vi "TestArmPathPlanner.vi"() -> ()   [LabVIEW 2017]
uses:
  ArgosLib/Path Planning/TypeDefs/Point2D.ctl
  General/MotionProfiling/TypeDefs/MotionProfileGeneratorParams.ctl
  <vilib>/Rock Robotics/WPI/ThirdParty/Phoenix-LabVIEW/Motor Controller/Controls/CTRE_Phoenix_MotorControl_TrajectoryPointTimeDur.ctl
  TypeDefs/RobotID.ctl
  General/MotionProfiling/TypeDefs/TrajectoryPoint.ctl
panel:
  out "Arm Rotation":T1(graph)
  out "Arm Extension":T1(graph)
  out "Overall Motion":T1(graph)
  out "TravelTime (s)":dbl
  in  "MotionProfileGeneratorParameters":T2={"Trajectory Point Interval (ms)"=40, "Maximum Travel Speed (units/s)"=110.0, "Velocity Ramp Time (ms)"=400.0, "Acceleration Ramp Time (ms)"=200.0} {"Acceleration Ramp Time (ms)" min=1.0; "Velocity Ramp Time (ms)" min=1.0; "Maximum Travel Speed (units/s)" min=0.0; "Trajectory Point Interval (ms)" items=["TrajectoryDuration_0ms"=0, "TrajectoryDuration_5ms"=5, "TrajectoryDuration_10ms"=10, "TrajectoryDuration_20ms"=20, "TrajectoryDuration_30ms"=30, "TrajectoryDuration_40ms"=40, "TrajectoryDuration_50ms"=50, "TrajectoryDuration_100ms"=100]}
  in  "EndPoint":T4={"X"=32.0, "Y"=50.0}
  in  "StartPoint":T4={"X"=32.0, "Y"=-45.0}
  in  "PathPointSpacing (in)":dbl=0.25
  in  "MaxArmLength":dbl=68.0
  in  "MinArmLength":dbl=44.0
  out "PathLength (in)":dbl
  out "NumPoints":i32
  out "Path":cluster{dbl[], dbl[]}[](graph)
  out "Update Rate (Hz)":dbl
  in  "stop":bool
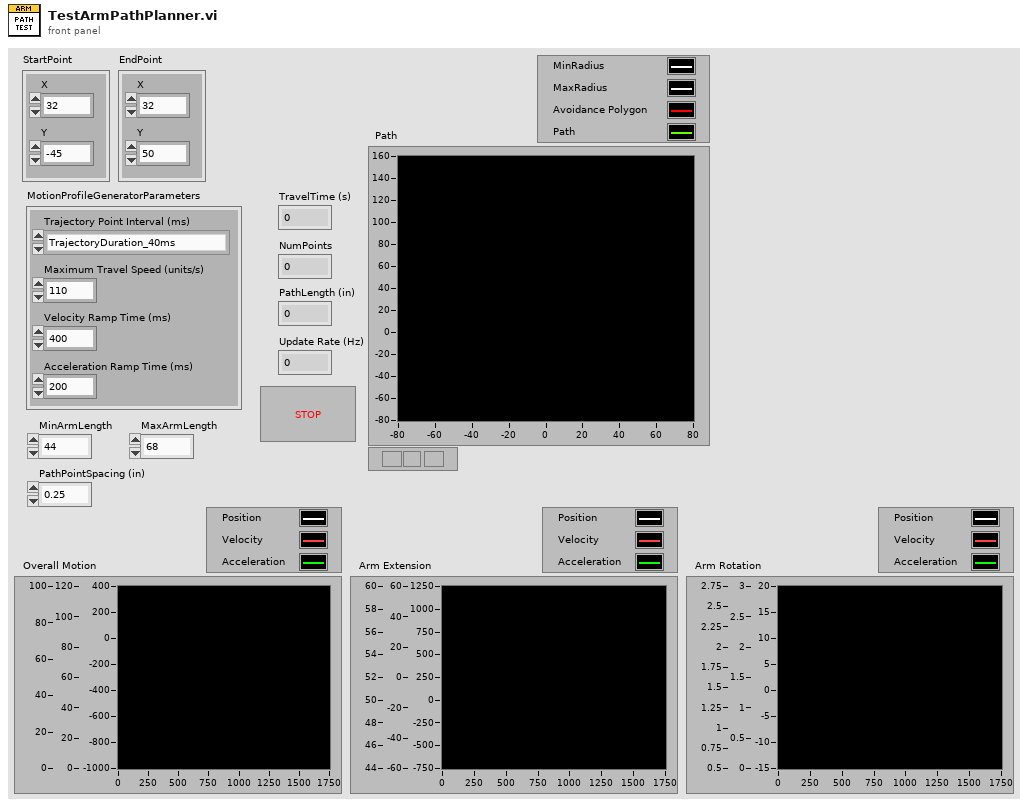
[diagram p1: front panel]
types:
  T1 = cluster{dbl, "Trajectory Point Interval (ms)":i32, dbl[][]}
  T2 = typedef "MotionProfileGeneratorParams.ctl" = cluster{"Trajectory Point Interval (ms)":T3, "Maximum Travel Speed (units/s)":dbl, "Velocity Ramp Time (ms)":dbl, "Acceleration Ramp Time (ms)":dbl}
  T3 = typedef "CTRE_Phoenix_MotorControl_TrajectoryPointTimeDur.ctl" = i32
  T4 = typedef "Point2D.ctl" = cluster{"X":dbl, "Y":dbl}
  T5 = typedef "RobotID.ctl" = enum16{"Competition", "Practice", "Programming", "Demo"}
  T6 = typedef "TrajectoryPoint.ctl" = cluster{"Position ":dbl, "Velocity ":dbl, "Time (ms)":T3, "Last Point":bool}
  T7 = typedef "Config_Robot.ctl" = cluster{"Motors":cluster{"DriveLeftPrimary":T8, "DriveLeftSecondary1":T8, "DriveRightPrimary":T8, "DriveRightSecondary1":T8, "RightIntake":T8, "LeftIntake":T8, "ArmPivot":T8, "ArmExtend":T8, "ArmPivot2":T8, "Climber":T8, "Selfie Stick":T8}, "Sensors":cluster{"IMU":T13, "LimitSwitch1":T15, "LimitSwitch2":T15, "BeamBreak":T15, "JeVois":T17}, "PID":cluster{"ArmExtend":T19, "ArmRotate":T19, "Drive":T19, "DriveGyro Kp ((in/sec)/deg)":dbl, "CameraPole":T19}, "Solenoids":cluster{"ArmClaw":T20, "IntakeExtend":T20, "IntakeOpen":T20, " Shifter":T20}, "RobotDimensions ":T22, "ArmHomePosition":T23, "SelfieStickParams":T24, "Enable Compressor":bool}
  T8 = typedef "Config_Motor.ctl" = cluster{"CAN Address":u8, "Invert":bool, "InvertSensor":bool, "Unit Conversion Factor":dbl, "Brake Mode":T9, "Reverse Limt Switch Mode":T10, "Forward Limt Swith Mode":T10, "PWM Channel":T11, "Motor Controller Type":T12}
  T9 = typedef "CTRE_Phoenix_MotorControl_NeutralMode.ctl" = enum8{"EEPROMSetting", "Override to Coast", "Override to Brake"}
  T10 = typedef "CTRE_Phoenix_MotorControl_LimitSwitchNormal.ctl" = enum16{"Normally Open", "Normally Closed", "Disabled"}
  T11 = typedef "FPGA_DIOPWMChannel.ctl" = enum8{"PWM 0", "PWM 1", "PWM 2", "PWM 3", "PWM 4", "PWM 5", "PWM 6", "PWM 7", "PWM 8", "PWM 9", "PWM MXP 0", "PWM MXP 1", "PWM MXP 2", "PWM MXP 3", "PWM MXP 4", "PWM MXP 5", "PWM MXP 6", "PWM MXP 7", "PWM MXP 8", "PWM MXP 9", "Invalid"}
  T12 = typedef "Config_MotorCtrlType.ctl" = enum16{"Disabled", "Talon SRX", "Talon SR"}
  T13 = typedef "Config_IMU.ctl" = cluster{"Yaw Axis":enum16{"X", "Y", "Z"}, "SPI Bus":T14, "AHRS Algorithm":enum16{"Complementary", "Madgwick"}, "Calibration Time (s)":dbl, "Calibrate On Open":bool}
  T14 = typedef "spi_bus.ctl" = enum16{"SPI On-Board, CS0", "SPI On-Board, CS1", "SPI On-Board, CS2", "SPI On-Board, CS3", "SPI MXP", "Invalid"}
  T15 = typedef "Config_DigitalIO.ctl" = cluster{"DIOChannel":T16, "Active Low":bool}
  T16 = typedef "FPGA_DIOChannel.ctl" = enum8{"DIO 0", "DIO 1", "DIO 2", "DIO 3", "DIO 4", "DIO 5", "DIO 6", "DIO 7", "DIO 8", "DIO 9", "DIO MXP 0", "DIO MXP 1", "DIO MXP 2", "DIO MXP 3", "DIO MXP 4", "DIO MXP 5", "DIO MXP 6", "DIO MXP 7", "DIO MXP 8", "DIO MXP 9", "DIO MXP 10", "DIO MXP 11", "DIO MXP 12", "DIO MXP 13", "DIO MXP 14", "DIO MXP 15", "SPI Port CS1", "SPI Port CS2", "SPI Port CS3", "SPI Port MISO", "SPI Port MOSI", "Invalid"}
  T17 = typedef "Config_SerialPort.ctl" = cluster{"Baud Rate":u32, "Parity":u16, "Data Bits":u16, "Stop Bits":u16, "Termination Char (0xA = '\\n' = LF)":u8, "Enable Termination Char? (T)":bool, "Flow Control":u16, "Timeout Value (ms)":u32, "Serial Port":T18}
  T18 = typedef "WPI_SerialPort.ctl" = enum16{"Onboard RS-232", "MXP TTL", "USB 1", "USB 2"}
  T19 = typedef "Config_PIDParams.ctl" = cluster{"P":dbl, "I":dbl, "D":dbl, "F":dbl, "IZone":dbl}
  T20 = typedef "Config_DoubleSolenoid.ctl" = cluster{"Forward Channel":T21, "Invert":bool, "Reverse Channel":T21}
  T21 = typedef "WPI_SolenoidChannel.ctl" = enum8{"Solenoid 0", "Solenoid 1", "Solenoid 2", "Solenoid 3", "Solenoid 4", "Solenoid 5", "Solenoid 6", "Solenoid 7", "Invalid"}
  T22 = typedef "Config_Dimensions.ctl" = cluster{"Length":dbl, "Height":dbl, "HeightOfBumpers":dbl, "DistanceFromFrameEdgeToPyramid ":dbl, "HeightOfFrameToIntake":dbl, "EdgeOfFrameToOrigin":dbl}
  T23 = typedef "Config_ArmHome.ctl" = cluster{"Angle (rad)":dbl, "Radius (in)":dbl}
  T24 = typedef "Config_SelfieStick.ctl" = cluster{"Home Height (in)":dbl, "CruiseVelocity":i32, "MaxAccel":i32, "Low Height (in)":dbl, "High Height (in)":dbl, "Mid Height (in)":dbl}
  T25 = typedef "Polygon2D.ctl" = T4[]
  T26 = typedef "ArmCoordinate.ctl" = cluster{"Radius (in)":dbl, "Angle (rad)":dbl}
  T27 = cluster{dbl, "Trajectory Point Interval (ms)":T3, dbl[][]}
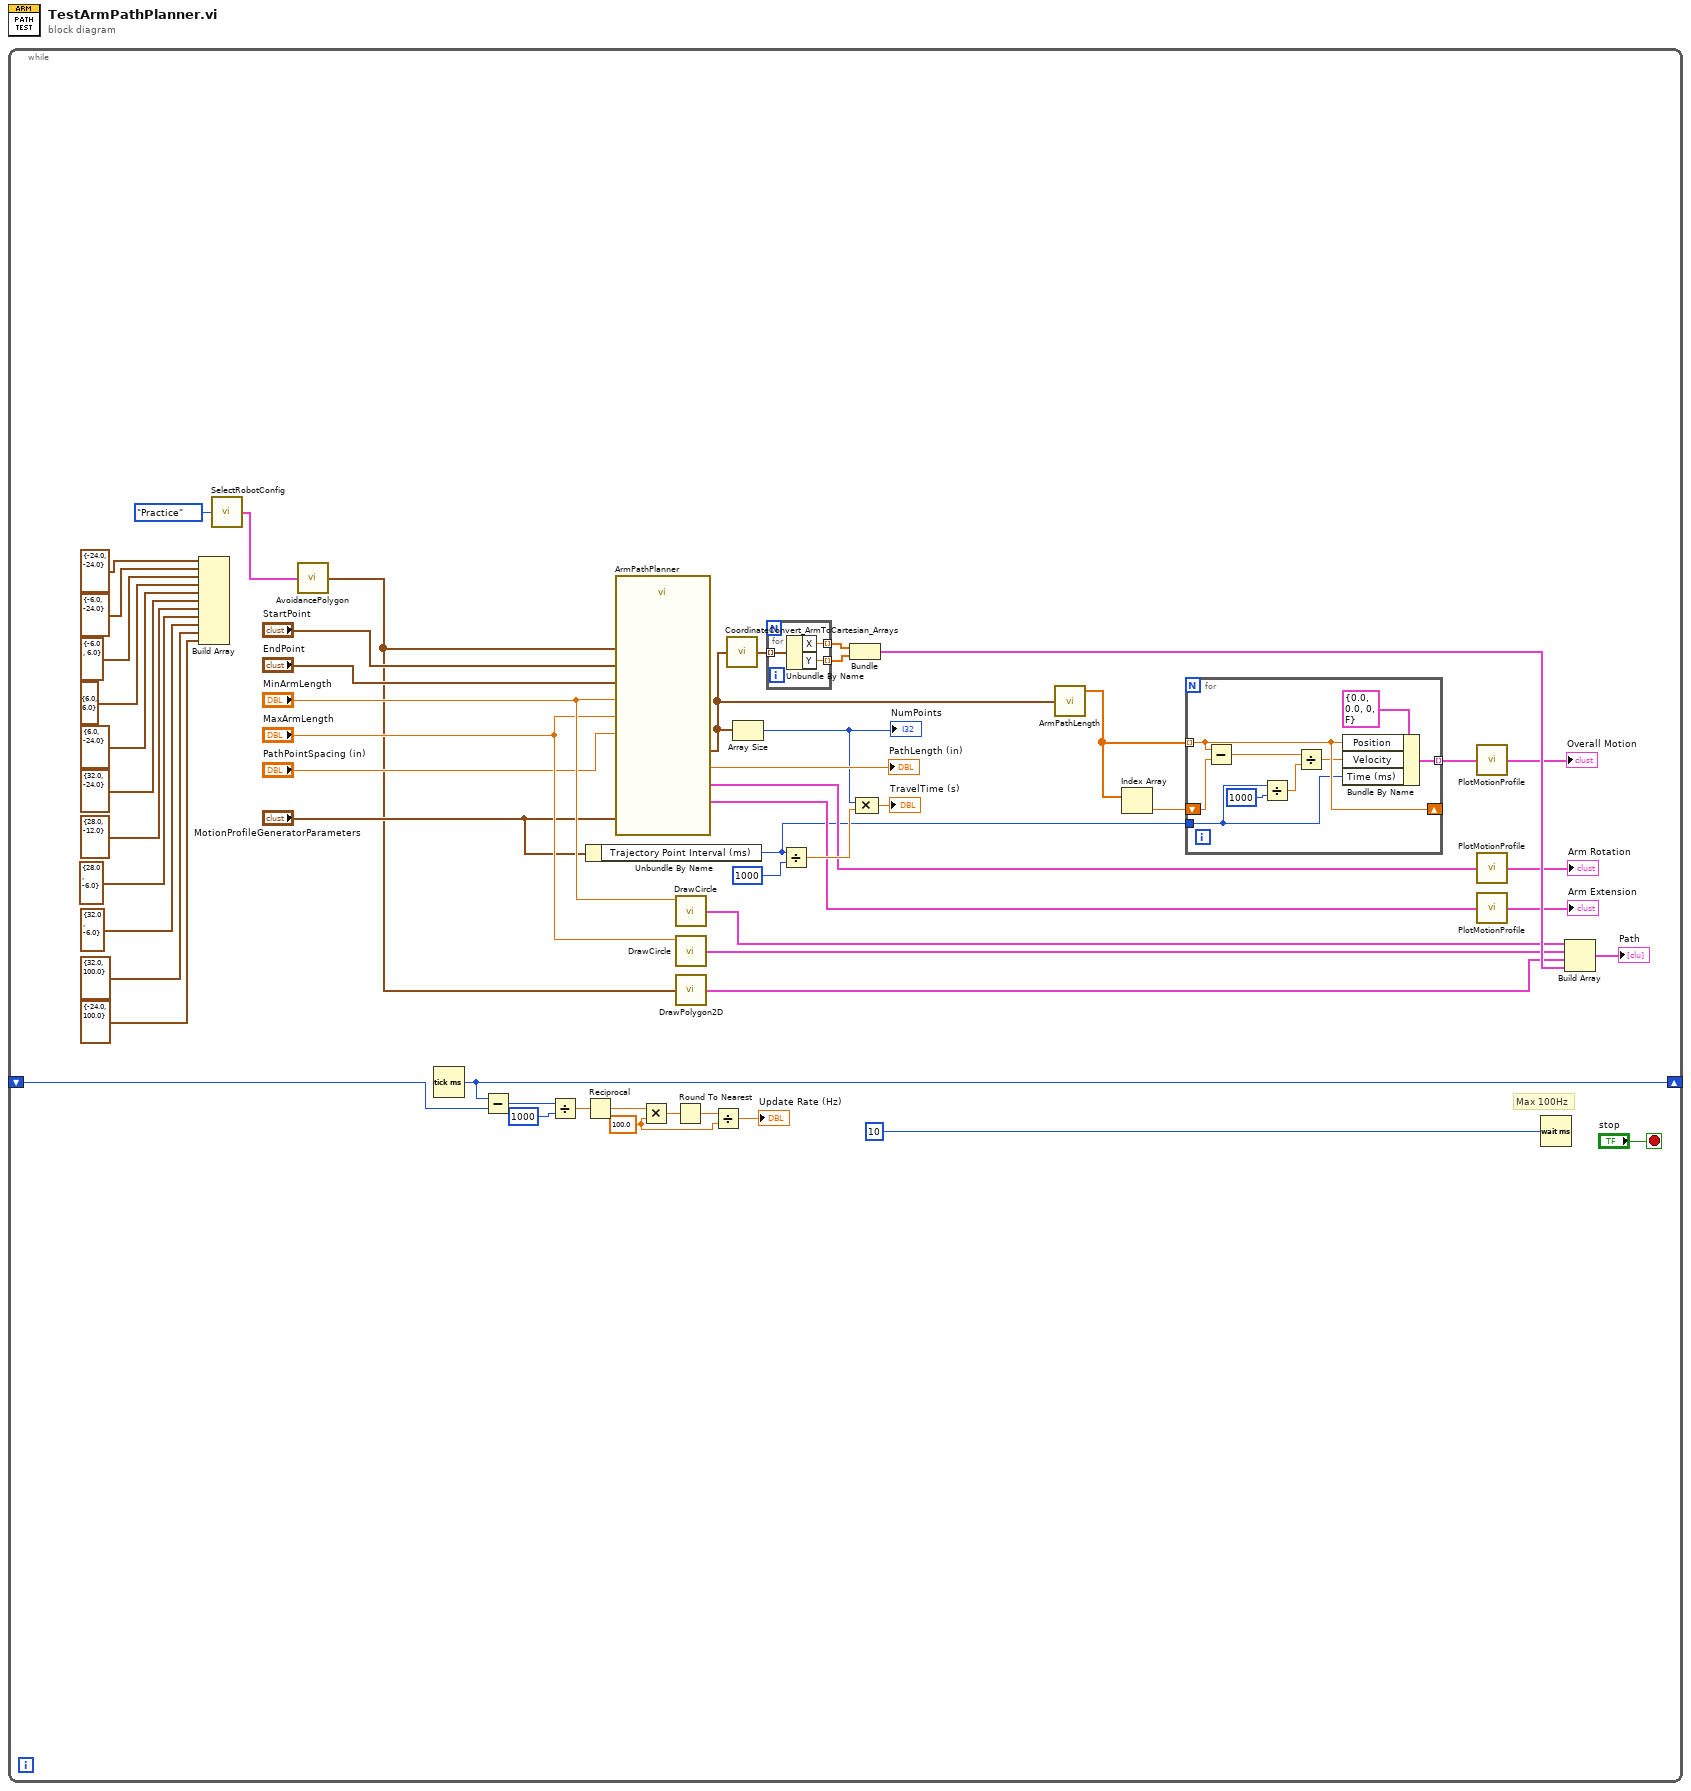
[diagram p0: block diagram]
diagram:
  n1 = while {
    shift-right: [w45] -> _
    shift-left: _ -> [w46]
    stop <- "stop" stop-if-true
    w48 = 100.0 ("y")
    # "Max 100Hz"
    n2 = Build Array(T4 {"X"=-24.0, "Y"=-24.0} ("2DPoint"), T4 {"X"=-6.0, "Y"=-24.0} ("2DPoint"), T4 {"X"=-6.0, "Y"=6.0} ("2DPoint"), T4 {"X"=6.0, "Y"=6.0} ("2DPoint"), T4 {"X"=6.0, "Y"=-24.0} ("2DPoint"), T4 {"X"=32.0, "Y"=-24.0} ("2DPoint"), T4 {"X"=28.0, "Y"=-12.0} ("2DPoint"), T4 {"X"=28.0, "Y"=-6.0} ("2DPoint"), T4 {"X"=32.0, "Y"=-6.0} ("2DPoint"), T4 {"X"=32.0, "Y"=100.0} ("2DPoint"), T4 {"X"=-24.0, "Y"=100.0} ("2DPoint")) -> ()  [unwired: 1 out]
    n3 = call "SelectRobotConfig.vi"("Robot ID"=RobotID."Practice") -> ("Selected Config"=w1:T7)
    n4 = call "AvoidancePolygon.vi"("RobotConfig"=w1) -> ("Polygon"=w3:T25)
    n5 = Tick Count (ms)() -> (millisecond timer value=w45:u32)
    n6 = Subtract(x=w45, y=w46) -> (x-y=w54:u32)
    n7 = Divide(x=w54, y=u32 1000) -> (x/y=w52:dbl)
    n8 = Reciprocal(x=w52) -> (1/x=w51:dbl)
    n9 = Unbundle By Name("MotionProfileGeneratorParameters") -> ("Trajectory Point Interval (ms)"=w7:T3)
    n10 = call "ArmPathPlanner.vi"("StartPoint"="StartPoint", "EndPoint"="EndPoint", "PathPointSpacing (in)"="PathPointSpacing (in)", "MinArmLength"="MinArmLength", "MaxArmLength"="MaxArmLength", "AvoidancePolygon"=w3, "MotionProfileGeneratorParameters"="MotionProfileGeneratorParameters") -> ("Path"=w8:T26[], "RotatePath"=w12:T6[], "ExtendPath"=w11:T6[], "PathLength (in)"=→"PathLength (in)":dbl)  [unwired: 9 in]
    n11 = Multiply(x=w51, y=w48) -> (x*y=w50:dbl)
    n12 = Round To Nearest(number=w50) -> (nearest integer value=w49:dbl)
    n13 = call "DrawCircle.vi"("Radius"="MinArmLength") -> ("Points"=w36:cluster{"X":dbl[], "Y":dbl[]})  [unwired: 3 in]
    n14 = call "DrawCircle.vi"("Radius"="MaxArmLength") -> ("Points"=w34:cluster{"X":dbl[], "Y":dbl[]})  [unwired: 3 in]
    n15 = call "DrawPolygon2D.vi"("Polygon"=w3) -> ("XYPlot"=w4:cluster{dbl[], dbl[]})
    n16 = Divide(x=w49, y=w48) -> (x/y=→"Update Rate (Hz)":dbl)
    n17 = call "CoordinateConvert_ArmToCartesian_Arrays.vi"("ArmCoordinates"=w8) -> ("XYPoints"=w42:T4[])
    n18 = Array Size(array=w8) -> (size(s)=w17:i32)
    "NumPoints" <- w17
    n19 = for {
      tunnel: w42 -> [w67] mode=indexing
      tunnel: [w66] -> w41 mode=indexing
      tunnel: [w65] -> w40 mode=indexing
      n20 = Unbundle By Name(w67) -> ("X"=w66:dbl, "Y"=w65:dbl)
    }
    n21 = Divide(x=w7, y=1000) -> (x/y=w15:dbl)
    n22 = Bundle(w41, w40) -> (w38:cluster{dbl[], dbl[]})  [unwired: 1 in]
    n23 = Compound Arithmetic op=MULTIPLY(w17, w15) -> (→"TravelTime (s)":dbl)
    n24 = call "ArmPathLength.vi"("ArmPathIn"=w8) -> ("IndexedPathLength"=w6:dbl[])  [unwired: 2 in, 2 out]
    n25 = Index Array(array=w6) -> (element=w5:dbl)  [unwired: 1 in]
    n26 = for {
      tunnel: [w63] -> w9 mode=indexing
      tunnel: w6 -> [w62] mode=indexing
      tunnel: w7 -> [w60]
      shift-right: [w62] -> _
      shift-left: w5 -> [w61]
      n27 = Subtract(x=w62, y=w61) -> (x-y=w58:dbl)
      n28 = Divide(x=w60, y=1000) -> (x/y=w57:dbl)
      n29 = Divide(x=w58, y=w57) -> (x/y=w56:dbl)
      n30 = Bundle By Name(cluster=T6 {"Position "=0.0, "Velocity "=0.0, "Time (ms)"=0, "Last Point"=FALSE} ("trajectory point"), "Position"=w62, "Velocity"=w56, "Time (ms)"=w60) -> (w63:T6)
    }
    n31 = call "PlotMotionProfile.vi"("Trajectory Points"=w9) -> ("MotionProfileGraph"=→"Overall Motion":T27)
    n32 = call "PlotMotionProfile.vi"("Trajectory Points"=w12) -> ("MotionProfileGraph"=→"Arm Rotation":T27)
    n33 = call "PlotMotionProfile.vi"("Trajectory Points"=w11) -> ("MotionProfileGraph"=→"Arm Extension":T27)
    n34 = Wait (ms)(milliseconds to wait=u32 10) -> ()  [unwired: 1 out]
    n35 = Build Array(w36, w34, w4, w38) -> (→"Path":cluster{"X":dbl[], "Y":dbl[]}[])
  }
